vi "MQTT Properties - Add Property.vi"(0 "Properties In":u8[](array[numeric]), 5 "Property Type":T1 items=["Payload Format Indicator"=1, "Message Expiry Interval"=2, "Content Type"=3, "Response Topic"=8, "Correlation Data"=9, "Subscription Identifier"=11, "Session Expiry Interval"=17, "Assigned Client Identifier"=18, "Server Keep Alive"=19, "Authentication Method"=21, "Authentication Data"=22, "Request Problem Information"=23, "Will Delay Interval"=24, "Request Response Information"=25, "Response Information"=26, "Server Reference"=28, "Reason String"=31, "Receive Maximum"=33, "Topic Alias Maximum"=34, "Topic Alias"=35, "Maximum QoS"=36, "Retain Available"=37, "User Property"=38, "Maximum Packet Size"=39, "Wildcard Subscription Available"=40, "Subscription Identifier Available"=41, "Shared Subscription Available"=42], 7 "Property Value":string) -> (4 "Properties Out":u8[](array[numeric]))   [LabVIEW 2019, in "KoRE-MQTT.lvlib"]
doc: "Copyright (c) 2025 KoRElibs.com\nSPDX-License-Identifier: EUPL-1.2\n\nThis VI is licensed under the European Union Public License (EUPL) Version 1.2. You may use this VI unmodified in proprietary works. If you distribute a modified version of this file, the modified file must be released under the EUPL-1.2. Full license: https://joinup.ec.europa.eu/asset/eupl/eupl/1.2/"
uses:
  KoRE-MQTT.lvlib
  TypeDefs/MQTT Property Type.ctl
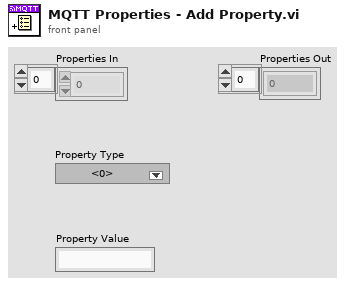
[diagram p1: front panel]
types:
  T1 = typedef "KoRE-MQTT.lvlib/MQTT Property Type.ctl" = u8
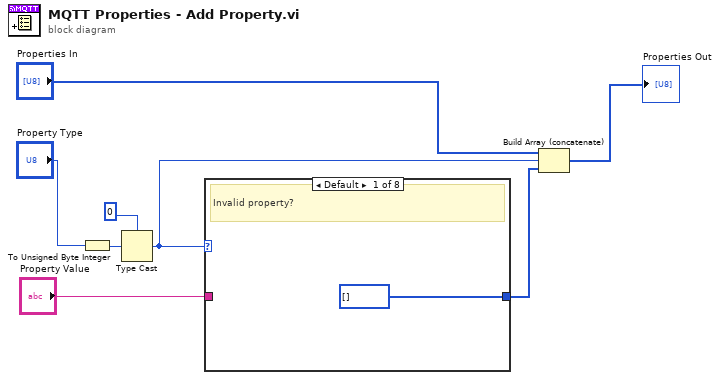
[diagram p0: block diagram]
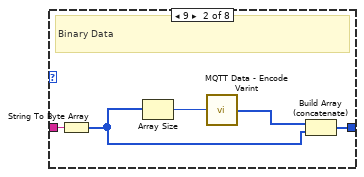
[diagram p2: hidden frame]
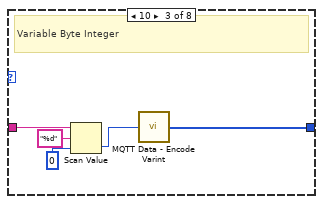
[diagram p3: hidden frame]
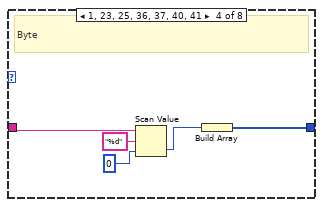
[diagram p4: hidden frame]
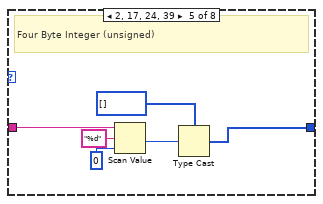
[diagram p5: hidden frame]
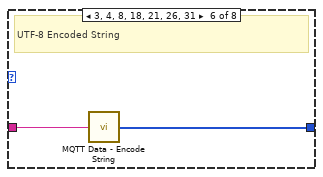
[diagram p6: hidden frame]
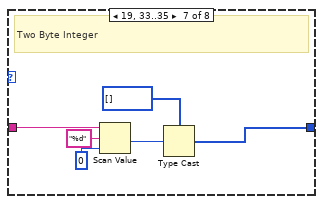
[diagram p7: hidden frame]
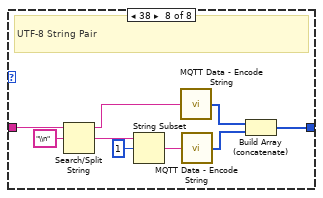
[diagram p8: hidden frame]
diagram:
  n1 = To Unsigned Byte Integer(number="Property Type") -> (unsigned 8bit integer=w4:T1)
  n2 = Type Cast(type=u8 0, x=w4) -> (*(type *) &x=w6:u8)
  n3 = case shown="Default" w6 {
    tunnel: "Property Value" -> [_ w14 w17 w23 w30 w32 w34 w47]
    tunnel: [u8[] [] ("Array") w10 w15 w22 w26 w31 w33 w39] -> w7
    frame Default {
      # "Invalid property?"
    }
    frame 9 {
      # "Binary Data"
      n4 = String To Byte Array(string=w14) -> (unsigned byte array=w11:u8[])
      n5 = Array Size(array=w11) -> (size(s)=w13:i32)
      n6 = call "MQTT Data - Encode Varint.vi"("Value"=w13) -> ("encoded value"=w12:u8[])  [unwired: 14 in]
      n7 = Build Array (concatenate)(w12, w11) -> (w10:u8[])
    }
    frame 10 {
      # "Variable Byte Integer"
      n8 = Scan Value(string=w17, format string="%d", default (0 dbl)=u32 0) -> (value=w16:u32)  [unwired: 1 out]
      n9 = call "MQTT Data - Encode Varint.vi"("Value"=w16) -> ("encoded value"=w15:u8[])  [unwired: 14 in]
    }
    frame 1, 23, 25, 36, 37, 40, 41 {
      # "Byte"
      n10 = Scan Value(string=w23, format string="%d", default (0 dbl)=u8 0) -> (value=w21:u8)  [unwired: 1 out]
      n11 = Build Array(w21) -> (w22:u8[])
    }
    frame 2, 17, 24, 39 {
      # "Four Byte Integer (unsigned)"
      n12 = Scan Value(string=w30, format string="%d", default (0 dbl)=u32 0) -> (value=w27:u32)  [unwired: 1 out]
      n13 = Type Cast(type=u8[] [], x=w27) -> (*(type *) &x=w26:u8[])
    }
    frame 3, 4, 8, 18, 21, 26, 31 {
      # "UTF-8 Encoded String"
      n14 = call "MQTT Data - Encode String.vi"("String in"=w32) -> ("Bytes out"=w31:u8[])  [unwired: 13 in, 1 out]
    }
    frame 19, 33..35 {
      # "Two Byte Integer"
      n15 = Scan Value(string=w34, format string="%d", default (0 dbl)=u16 0) -> (value=w36:u16)  [unwired: 1 out]
      n16 = Type Cast(type=u8[] [], x=w36) -> (*(type *) &x=w33:u8[])
    }
    frame 38 {
      # "UTF-8 String Pair"
      n17 = Search/Split String(string=w47, search string/char (-)="\\n") -> (substring before match=w43:string, match + rest of string=w45:string)  [unwired: 1 in, 1 out]
      n18 = String Subset(string=w45, offset (0)=1) -> (substring=w42:string)  [unwired: 1 in]
      n19 = call "MQTT Data - Encode String.vi"("String in"=w43) -> ("Bytes out"=w41:u8[])  [unwired: 13 in, 1 out]
      n20 = call "MQTT Data - Encode String.vi"("String in"=w42) -> ("Bytes out"=w40:u8[])  [unwired: 13 in, 1 out]
      n21 = Build Array (concatenate)(w41, w40) -> (w39:u8[])
    }
  }
  n22 = Build Array (concatenate)("Properties In", w6, w7) -> (→"Properties Out":u8[])
